vi "GenerateListOfSuccessSpecsOrPreviewOrder.vi"(8 "error in (no error)":errorcluster, 9 "Generated file":T2, 11 "SolutionBuilder in":refnum<class "SolutionBuilder.lvclass">) -> (0 "error out":errorcluster, 1 "Builds":T1[](array[typedef]), 3 "SolutionBuilder out":refnum<class "SolutionBuilder.lvclass">)   [LabVIEW 2019, in "SolutionBuilder.lvlib" / "SolutionBuilder.lvclass"]
uses:
  SolutionBuilder.lvclass
  BuildManager/GeneratedFile.ctl
  BuildManager/BuildProjectInfo.ctl
  ProjectItem/ProjectItem.lvclass
  BuildManager/BuildManager.lvclass
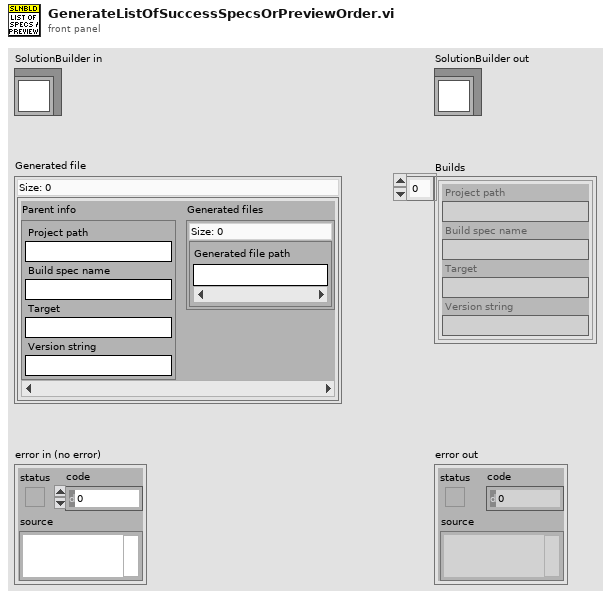
[diagram p1: front panel]
types:
  T1 = typedef "SolutionBuilder.lvlib/BuildManager.lvclass/BuildProjectInfo.ctl" = cluster{"Project path":string, "Build spec name":string, "Target":string, "Version string":string}
  T2 = typedef "SolutionBuilder.lvlib/BuildManager.lvclass/GeneratedFile.ctl" = map{T1, set{string}}
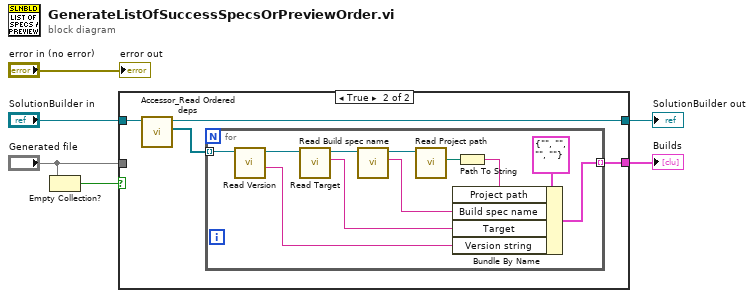
[diagram p0: block diagram]
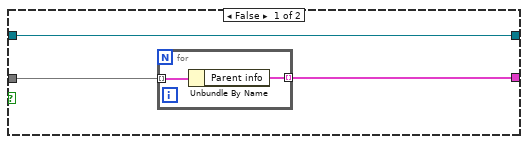
[diagram p2: hidden frame]
diagram:
  n1 = Empty Collection?(1:"Generated file") -> (0:w4:bool)
  n2 = case shown="True" w4 {
    tunnel: "Generated file" -> [w9 _]
    tunnel: [w8 w13] -> w3
    tunnel: "SolutionBuilder in" -> [w8 w14]
    tunnel: [w7 w12] -> w1
    frame False {
      n3 = for {
        tunnel: w9 -> [w11] mode=indexing
        tunnel: [w10] -> w7 mode=indexing
        n4 = Unbundle By Name(w11) -> ("Parent info"=w10:T1)
      }
    }
    frame True {
      n5 = call "Accessor_Read Ordered deps.vi"("SolutionBuilder in"=w14) -> ("Ordered deps"=w15:refnum<class "ProjectItem.lvclass">[], "SolutionBuilder out"=w13:refnum<class "SolutionBuilder.lvclass">)  [unwired: 8 in, 1 out]
      n6 = for {
        tunnel: w15 -> [w23] mode=indexing
        tunnel: [w19] -> w12 mode=indexing
        n7 = call "Read Version.vi"("ProjectItem in"=w23) -> ("Version string"=w16:string, "ProjectItem out"=w22:refnum<class "ProjectItem.lvclass">)  [unwired: 8 in, 1 out]
        n8 = call "Read Target.vi"("ProjectItem in"=w22) -> ("Target"=w17:string, "ProjectItem out"=w24:refnum<class "ProjectItem.lvclass">)  [unwired: 9 in]
        n9 = call "Read Build spec name.vi"("ProjectItem in"=w24) -> ("Build spec name"=w18:string, "ProjectItem out"=w26:refnum<class "ProjectItem.lvclass">)  [unwired: 9 in]
        n10 = call "Read Project path.vi"("ProjectItem in"=w26) -> ("Project path"=w25:path)  [unwired: 9 in, 1 out]
        n11 = Path To String(path=w25) -> (string=w20:string)
        n12 = Bundle By Name(cluster=T1 {"Project path"="", "Build spec name"="", "Target"="", "Version string"=""} ("Parent info"), "Project path"=w20, "Build spec name"=w18, "Target"=w17, "Version string"=w16) -> (w19:T1)
      }
    }
  }
  "SolutionBuilder out" <- w3
  "Builds" <- w1
  "error out" <- "error in (no error)"
